vi "VM3 - Arbitrary Data.vi"(5 "cmd (read)":enum16{"create", "destroy", "write", "read"}(ring)=enum."read", 6 "var type in":u32=128, 7 "VC Handle":T2, 8 "error in":errorcluster, 9 "writer ID":u32, 10 "flattened value in":string, 11 "name_spec":string) -> (0 "error out":errorcluster, 1 "stats":T1, 2 "flattened value out":string, 3 "dup name_spec":string, 4 "var type out":u32)   [LabVIEW 2021]
doc: "This VI manages variables that can have an arbitrary data type, supporting both predefined and user-defined data types. Variable values are represented in the Flattened-To-String format, with the exception of the String data type, which uses the native LabVIEW string representation. For predefined data types, the VI checks the consistency of the data type code and value format, returning an error in the event of a mismatch. Refer to the VI Help for more details.\n\n<b>cmd</b> specifies the operation to perform on the variable: create, write, read, or destroy.\n\n<b>VC Handle</b> specifies the handle of the variable context. To operate on a global variable, pass -1 to this input. <b>name_spec</b> is the name specifier of the desired variable; usually, it is merely a variable name (see the VI Help for more options).\n\n<b>flattened value in</b> and <b>flattened value out</b> are the input and output values written to or read from the variable, respectively.\n\n<b>writer ID</b> specifies the Writer ID to be set along with the new value when writing or creating a variable.\n\n<b>stats</b> returns information about the most recent value of the variable, such as Writer ID, update time, and update counter.\n\n<b>var type</b> specifies the data type code of the target variable. VarMan strictly checks this data type code to ensure it matches the variable data type. However, passing -1 to this input allows reading a variable value of an arbitrary data type, in which case the <b>var type out</b> indicator returns the actual data type code. Passing -1 to this control during write or create operations causes the VI to return an error.\n\n::: CalcExpress Toolkit :::\nCopyright (c) 2000-2026 Konstantin Shifershteyn. All rights reserved."
uses:
  cetypes.llb/VarMan Variable Context Handle.ctl
  cetypes.llb/VarMan Variable Data Statistics.ctl
  cetypes.llb/VarMan Error Code.ctl
  cersrc/celveng32.dll
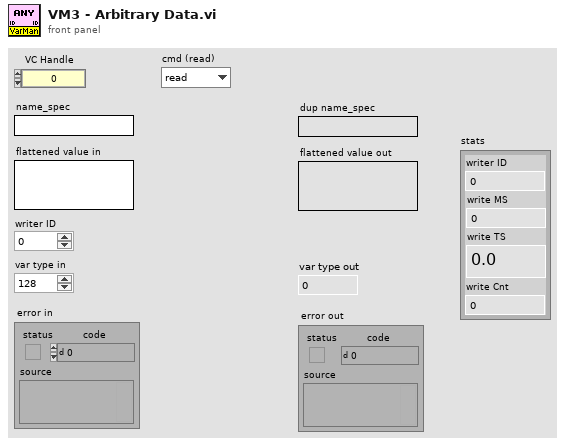
[diagram p1: front panel]
types:
  T1 = typedef "VarMan Variable Data Statistics.ctl" = cluster{"writer ID":u32, "write MS":u32, "write TS":dbl, "write Cnt":u32}
  T2 = typedef "VarMan Variable Context Handle.ctl" = i32
  T3 = typedef "VarMan Error Code.ctl" = u16
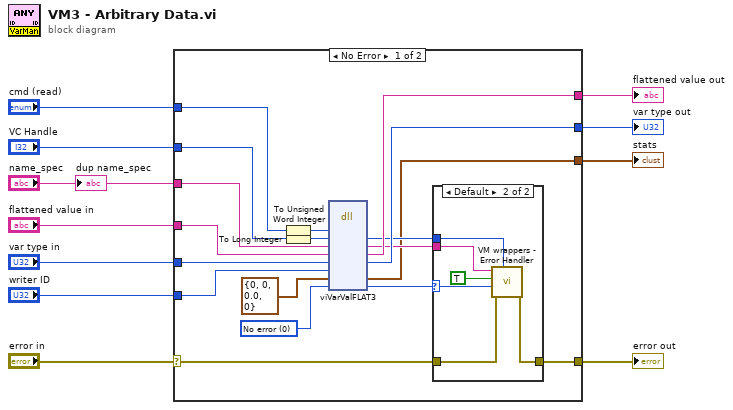
[diagram p0: block diagram]
diagram:
  n1 = case shown="No Error" "error in" {
    selector: "error in" -> [w17 w39]
    tunnel: [w29 w39] -> w11
    tunnel: "flattened value in" -> [w28 w38]
    tunnel: "var type in" -> [w27 w37]
    tunnel: [w26 w37] -> w8
    tunnel: "name_spec" -> [w25 _]
    tunnel: "VC Handle" -> [w24 _]
    tunnel: [w23 w38] -> w5
    tunnel: "writer ID" -> [w22 _]
    tunnel: "cmd (read)" -> [w16 _]
    tunnel: [w12 _] -> w1
    frame No Error {
      w21 = T3 0 items=["No error", "Invalid variable type", "Variable not found", "Variable already exists", "Invalid context handle", "Input error", "Invalid data format", "No history attached", "History already attached", "Invalid history parameters", "Wrong variable name", "Wrong alias name", "Non-unique alias", "Alias not found", "No alias associated", "Alias already associated", "Wrong context name", "Non-unique context name", "Context name not found", "Invalid parameter", "Generic error", "Memory Full", "Unrecognized LV error", "Unknown error code"] ("VarMan error")
      n2 = To Unsigned Word Integer(number=w16) -> (unsigned 16bit integer=w15:u16)
      n3 = To Long Integer(number=w24) -> (32bit integer=w14:T2)
      n4 = dll-call lib="C:/LV Projects/CalcExpress 40 LV2021/vi.lib/addons/CalcExpress/cersrc/celveng*.dll" fn="viVarValFLAT3"("cmd"=w15, "vch"=w14, "name"=w25, "val"=w28, "type"=w27, "writerID"=w22, "wrStats"=T1 {"writer ID"=0, "write MS"=0, "write TS"=0.0, "write Cnt"=0} ("stats"), "errc"=w21) -> ("vch"=w18:i32, "name"=w19:string, "val"=w23:string, "type"=w26:u32, "wrStats"=w12:T1, "errc"=w20:T3)  [unwired: 6 in, 2 out]
      n5 = case shown="Default" w20 {
        selector: w20 -> [_ w33]
        tunnel: [w30 w36] -> w29
        tunnel: w17 -> [w30 w35]
        tunnel: w19 -> [_ w32]
        tunnel: w18 -> [_ w31]
        frame 0 {
        }
        frame Default {
          n6 = call "VM wrappers - Error Handler.vi"("VC Handle"=w31, "error before"=w35, "VarMan error"=w33, "show name spec (F)"=TRUE, "name spec"=w32) -> ("error out"=w36:errorcluster)  [unwired: 5 in, 1 out]
        }
      }
    }
    frame Error {
    }
  }
  "error out" <- w11
  "flattened value out" <- w5
  "var type out" <- w8
  "stats" <- w1
  "dup name_spec" <- "name_spec"
